vi "invknode_config.vi"() -> ()   [LabVIEW 2014]
panel:
  in  "Invoke Node Class Name":string
  in  "error in (no error)":errorcluster
  in  "reference":refnum<vi>
  out "error out":errorcluster
  out "reference out":refnum<vi>
  in  "Allow Alternate Names? (F)":bool
  in  "ID String":string
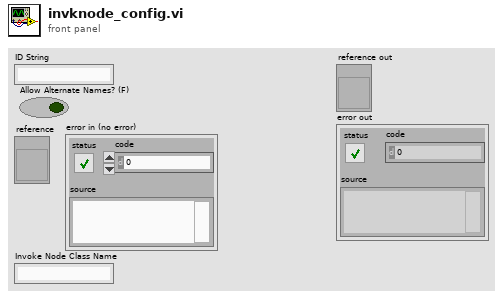
[diagram p1: front panel]
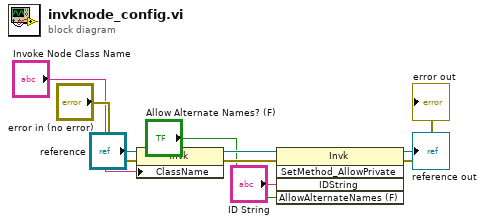
[diagram p0: block diagram]
diagram:
  n1 = property class="Invk"(reference="reference", error in="error in (no error)", "ClassName"="Invoke Node Class Name") -> (reference out=w9:refnum<vi>, error out=w8:errorcluster)
  n2 = invoke class="Invk" method="SetMethod_AllowPrivate"(reference=w9, error in=w8, "IDString"="ID String", "AllowAlternateNames (F)"="Allow Alternate Names? (F)") -> (reference out=→"reference out":refnum<vi>, error out=→"error out":errorcluster)  [unwired: 1 in, 3 out]
